vi "Sous_VI_RT_Virage.vi"(8 "Erreur in":errorcluster caption="Erreur", 10 "Compteur IN":i32, 11 "Etat IN":T1=enum."Tourner") -> (0 "Erreur out":errorcluster caption="Erreur", 1 "Information de fin de process":bool, 2 "Compteur OUT":i32, 3 "Etat OUT":T1=enum."Tourner", 5 "Detection suiveur de ligne":bool[](array[boolean]))   [LabVIEW 2018]
doc: "Effectue une rotation dans le sens horaire jusqu'à détecter une ligne"
uses:
  enum_RT_Virage.ctl
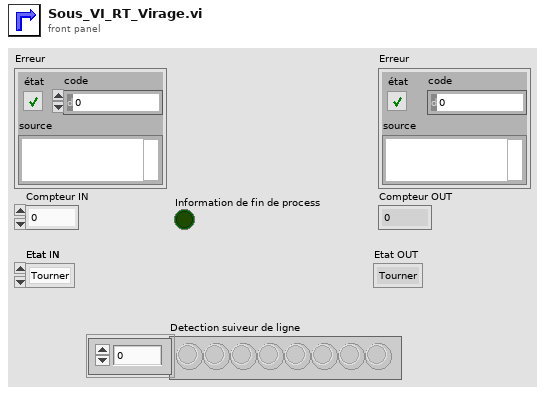
[diagram p1: front panel]
types:
  T1 = typedef "enum_RT_Virage.ctl" = enum16{"Avancer", "STOP", "Lacher Ligne", "Tourner"}
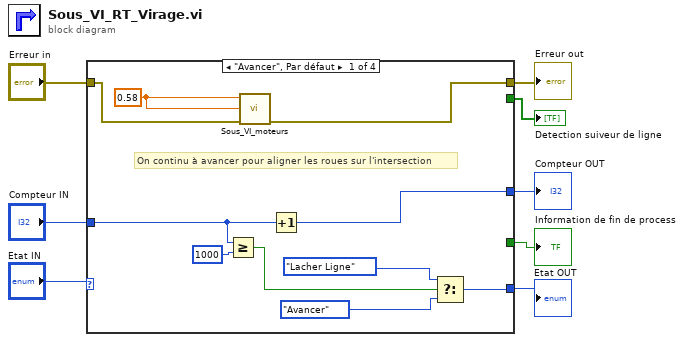
[diagram p0: block diagram]
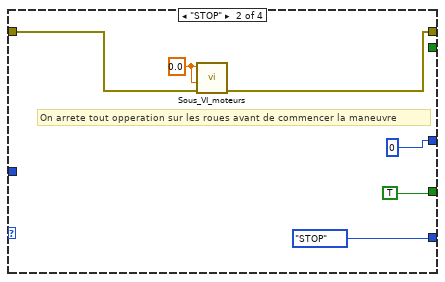
[diagram p2: hidden frame]
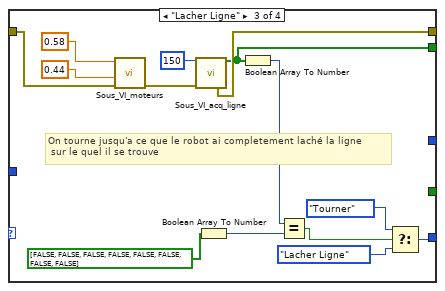
[diagram p3: hidden frame]
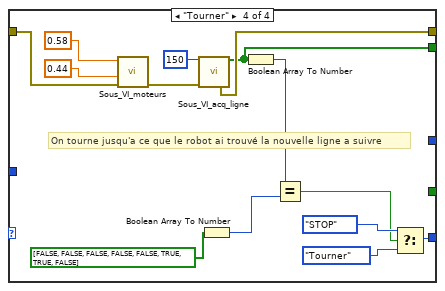
[diagram p4: hidden frame]
diagram:
  n1 = case shown="\"Avancer\", Par défaut" "Etat IN" {
    tunnel: [w16 enum_RT_Virage."STOP" w32 w39] -> w1
    tunnel: "Erreur in" -> [w10 w23 w33 w45]
    tunnel: [w9 w22 w30 w44] -> w7
    tunnel: [w15 0 _ _] -> w5
    tunnel: "Compteur IN" -> [w14 _ _ _]
    tunnel: [_ _ w27 w43] -> w4
    tunnel: [_ TRUE _ _] -> w3
    frame "Avancer", Default {
      w11 = 0.58
      # "On continu à avancer pour aligner les roues sur l'intersection"
      n2 = Greater Or Equal?(x=w14, y=1000) -> (x >= y?=w17:bool)
      n3 = call "Sous_VI_moteurs.vi"("error in (no error)"=w10, "Moteur Droit"=w11, "Moteur Gauche"=w11) -> ("error out"=w9:errorcluster)  [unwired: 8 in]
      n4 = Increment(x=w14) -> (x+1=w15:i32)
      n5 = Select(t=enum_RT_Virage."Lacher Ligne", s=w17, f=enum_RT_Virage."Avancer") -> (s? t:f=w16:T1)
    }
    frame "STOP" {
      w24 = 0.0 ("Moteur Gauche")
      # "On arrete tout opperation sur les roues avant de commencer la maneuvre"
      n6 = call "Sous_VI_moteurs.vi"("error in (no error)"=w23, "Moteur Droit"=w24, "Moteur Gauche"=w24) -> ("error out"=w22:errorcluster)  [unwired: 8 in]
    }
    frame "Lacher Ligne" {
      # "On tourne jusqu'a ce que le robot ai completement laché la ligne\n sur le quel il se trouve"
      n7 = call "Sous_VI_moteurs.vi"("error in (no error)"=w33, "Moteur Droit"=0.44 ("moteur droit lent"), "Moteur Gauche"=0.58 ("moteur gauche vite")) -> ("error out"=w35:errorcluster)  [unwired: 8 in]
      n8 = call "Sous_VI_acq_ligne.vi"("Seuil"=150, "error in (no error)"=w35) -> ("x > y ?"=w27:bool[], "error out"=w30:errorcluster)  [unwired: 8 in, 4 out]
      n9 = Boolean Array To Number(Boolean array=bool[] [FALSE, FALSE, FALSE, FALSE, FALSE, FALSE, FALSE, FALSE]) -> (number=w38:u32)
      n10 = Boolean Array To Number(Boolean array=w27) -> (number=w37:u32)
      n11 = Equal?(x=w37, y=w38) -> (x = y?=w31:bool)
      n12 = Select(t=enum_RT_Virage."Tourner", s=w31, f=enum_RT_Virage."Lacher Ligne") -> (s? t:f=w32:T1)
    }
    frame "Tourner" {
      # "On tourne jusqu'a ce que le robot ai trouvé la nouvelle ligne a suivre"
      n13 = call "Sous_VI_moteurs.vi"("error in (no error)"=w45, "Moteur Droit"=0.44 ("moteur droit lent"), "Moteur Gauche"=0.58 ("moteur gauche vite")) -> ("error out"=w49:errorcluster)  [unwired: 8 in]
      n14 = call "Sous_VI_acq_ligne.vi"("Seuil"=150, "error in (no error)"=w49) -> ("x > y ?"=w43:bool[], "error out"=w44:errorcluster)  [unwired: 8 in, 4 out]
      n15 = Boolean Array To Number(Boolean array=bool[] [FALSE, FALSE, FALSE, FALSE, FALSE, TRUE, TRUE, FALSE]) -> (number=w52:u32)
      n16 = Boolean Array To Number(Boolean array=w43) -> (number=w51:u32)
      n17 = Equal?(x=w51, y=w52) -> (x = y?=w40:bool)
      n18 = Select(t=enum_RT_Virage."STOP", s=w40, f=enum_RT_Virage."Tourner") -> (s? t:f=w39:T1)
    }
  }
  "Erreur out" <- w7
  "Compteur OUT" <- w5
  "Detection suiveur de ligne" <- w4
  "Information de fin de process" <- w3
  "Etat OUT" <- w1
